vi "lvmcp_staticviinfo.vi"() -> ()   [LabVIEW 2026]
panel:
  out "error out":errorcluster
  out "strict":bool
  out "path":path
  in  "reference":refnum<vi>
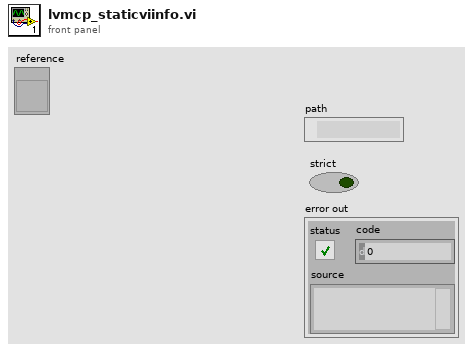
[diagram p1: front panel]
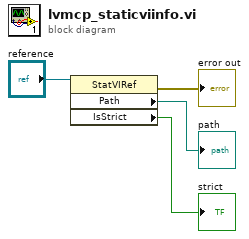
[diagram p0: block diagram]
diagram:
  n1 = property class="StatVIRef"(reference="reference") -> (error out=→"error out":errorcluster, "Path"=→"path":path, "IsStrict"=→"strict":bool)  [unwired: 1 in, 1 out]
